vi "AddChildtoNode.vi"(8 "error in":errorcluster, 10 "child in":T1, 11 "Engine Parent Editor Node in":refnum<class "Engine Parent Editor Node.lvclass">) -> (0 "error out":errorcluster, 3 "Engine Parent Editor Node out":refnum<class "Engine Parent Editor Node.lvclass">)   [LabVIEW 2014, in "PL Framework Configuration Tool.lvlib" / "Engine Parent Editor Node.lvclass"]
uses:
  Engine Parent Editor Node.lvclass
  <vilib>/NI/Configuration Framework/Node/NodeRef.ctl
  <vilib>/NI/Configuration Framework/Node/NISE_CEF_Node.lvclass
  <vilib>/NI/Configuration Framework/serializable node/NISE_CEF_serializable node.lvclass
  Targets/Targets.lvclass
  <vilib>/NI/Configuration Framework/Node/NISE_CEF_Node.lvclass/NISE_CEF_Node.ctl
  <vilib>/NI/Configuration Framework/serializable configuration/NISE_CEF_serializable configuration.lvclass/NISE_CEF_serializable configuration.ctl
  Targets/Targets.lvclass/Targets.ctl
  Targets/Read Configuration Class Name.vi
  Targets/Write Configuration Class Name.vi
  <vilib>/Utility/LVClass/Get LV Class Name.vi
  <vilib>/NI/Configuration Framework/error generator/NISE_error generator.vi
  read engine configuration.vi
  write engine configuration.vi
  <vilib>/NI/Configuration Framework/serializable configuration/NISE_CEF_serializable configuration.lvclass
  <vilib>/NI/Module Execution Interface/Engine Configuration/engine configuration.lvclass
  TBM Configuration Node/TBM Configuration Node.lvclass
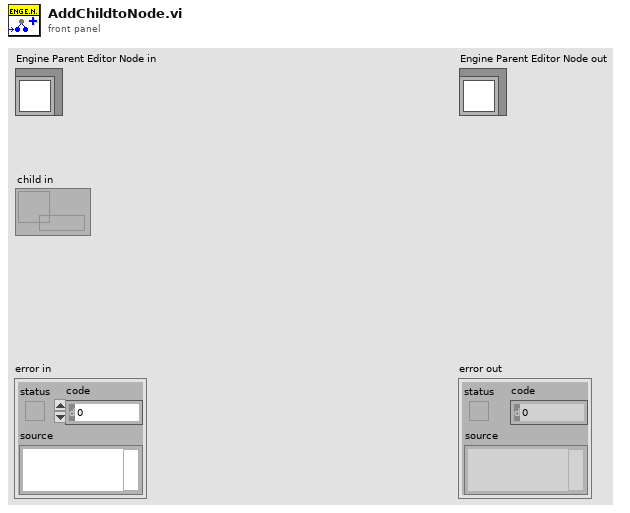
[diagram p1: front panel]
types:
  T1 = typedef "NISE_CEF_Node.lvclass/NodeRef.ctl" = refnum<data-value>
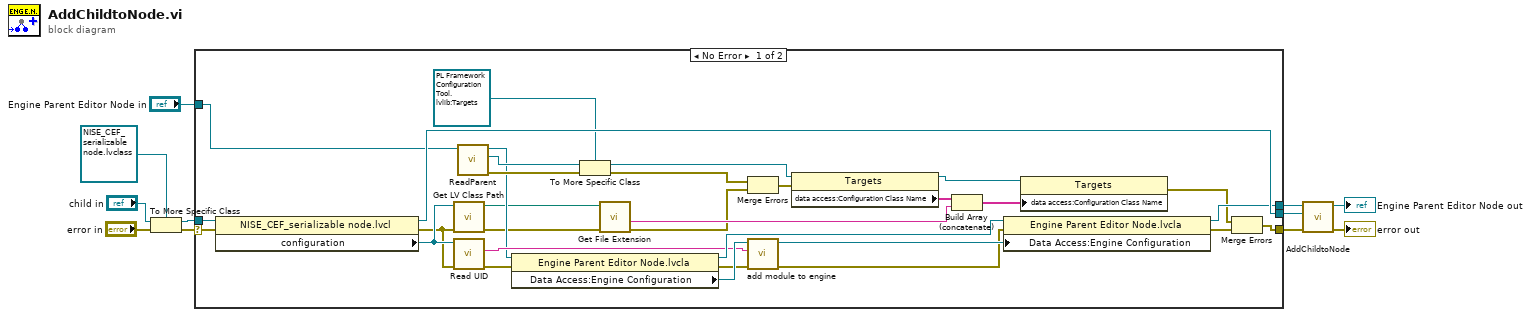
[diagram p0: block diagram]
diagram:
  n1 = To More Specific Class(target class=refnum<data-value> refnum, reference="child in", error in="error in") -> (specific class reference=w8:refnum<data-value>, error out=w6:errorcluster)
  n2 = case shown="No Error" w6 {
    selector: w6 -> [w40 w44]
    tunnel: [w12 w44] -> w5
    tunnel: [w42 w43] -> w9
    tunnel: w8 -> [w41 w43]
    tunnel: "Engine Parent Editor Node in" -> [w27 w45]
    tunnel: [w38 w45] -> w1
    frame No Error {
      n3 = property class="NISE_CEF_serializable node.lvcl"(reference=w41, error in=w40) -> (reference out=w42:refnum<data-value>, error out=w18:errorcluster, "configuration"=w22:refnum<class "NISE_CEF_serializable configuration.lvclass">)
      n4 = call <vilib>:"Get LV Class Path.vi"("error in (no error)"=w18, "object"=w22) -> ("error out"=w21:errorcluster, "class path"=w20:path)  [unwired: 8 in]
      n5 = call <vilib>:"Read UID.vi"("error in"=w18, "configuration in"=w22) -> ("error out"=w39:errorcluster, "instance id"=w32:string)  [unwired: 7 in, 1 out]
      n6 = call <vilib>:"ReadParent.vi"("node in"=w27) -> ("error out"=w30:errorcluster, "parent"=w28:T1, "node out"=w26:refnum<class "Engine Parent Editor Node.lvclass">)  [unwired: 8 in]
      n7 = property class="Engine Parent Editor Node.lvcla"(reference=w26, error in=w39) -> (reference out=w37:refnum<class "Engine Parent Editor Node.lvclass">, error out=w33:errorcluster, "Data Access:Engine Configuration"=w36:refnum<class "engine configuration.lvclass">)
      n8 = To More Specific Class(target class=refnum<data-value> refnum, reference=w28, error in=w30) -> (specific class reference=w29:refnum<data-value>, error out=w16:errorcluster)
      n9 = call <vilib>:"Get File Extension.vi"("error in (no error)"=w21, "file"=w20) -> ("error out"=w17:errorcluster, "filename without extension"=w19:string)  [unwired: 6 in, 2 out]
      n10 = Merge Errors(w16, w17) -> (w15:errorcluster)
      n11 = call-dynamic "add module to engine.vi"("error in"=w33, "module ID"=w32, "engine configuration in"=w36) -> ("error out"=w34:errorcluster, "engine configuration out"=w35:refnum<class "engine configuration.lvclass">)  [unwired: 7 in]
      n12 = property class="Targets"(reference=w29, error in=w15) -> (reference out=w25:refnum<data-value>, "data access:Configuration Class Name"=w24:string[])  [unwired: 1 out]
      n13 = Build Array (concatenate)(w24, w19) -> (w23:string[])
      n14 = property class="Engine Parent Editor Node.lvcla"(reference=w37, error in=w34, "Data Access:Engine Configuration"=w35) -> (reference out=w38:refnum<class "Engine Parent Editor Node.lvclass">, error out=w13:errorcluster)
      n15 = property class="Targets"(reference=w25, "data access:Configuration Class Name"=w23) -> (error out=w14:errorcluster)  [unwired: 1 in, 1 out]
      n16 = Merge Errors(w14, w13) -> (w12:errorcluster)
    }
    frame Error {
    }
  }
  n17 = call-parent "AddChildtoNode.vi"("error in"=w5, "child in"=w9, "NISE_CEF_Node in"=w1) -> ("error out"=→"error out":errorcluster, "NISE_CEF_Node out"=→"Engine Parent Editor Node out":refnum<class "Engine Parent Editor Node.lvclass">)  [unwired: 7 in]
